vi "Get Class Plugin Parent.vi"(8 "error in (no error)":errorcluster, 11 "LV Class Path":path) -> (0 "error out":errorcluster, 1 "object":refnum<class>, 2 "Qualified Name":string, 3 "Valid":bool)   [LabVIEW 2021, in "Channel.lvlib"]
uses:
  Channel.lvlib
  Channel/Channel_class/Channel.lvclass
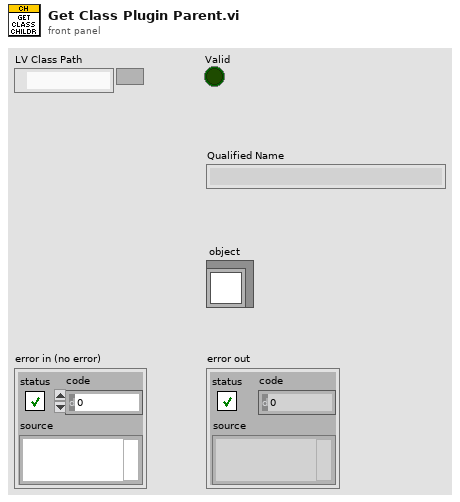
[diagram p1: front panel]
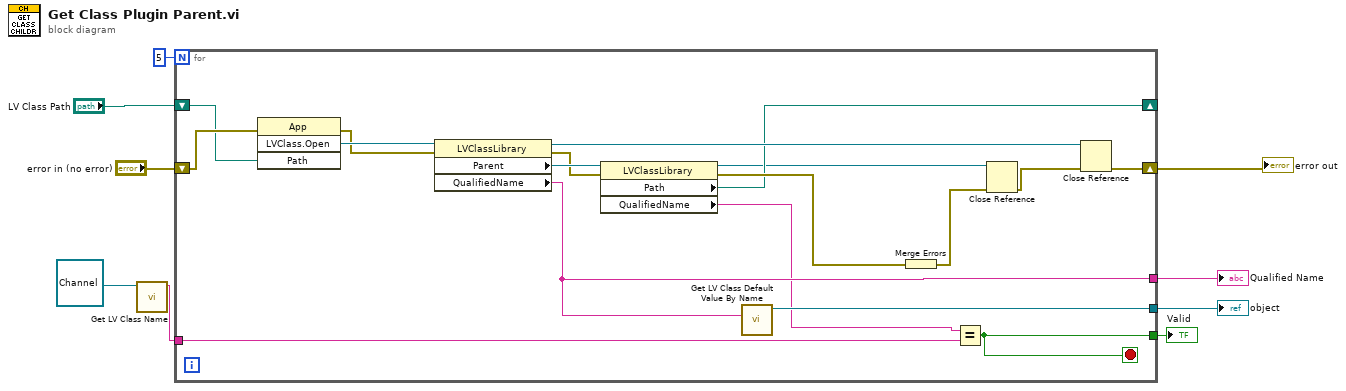
[diagram p0: block diagram]
diagram:
  n1 = call <vilib>:"Get LV Class Name.vi"("object"=refnum<class "Channel.lvclass"> refnum ("Channel.lvlib:Channel")) -> ("class name"=w3:string)  [unwired: 9 in, 1 out]
  n2 = for {
    N: 5 -> [_]
    tunnel: [w11] -> w7
    tunnel: [w16] -> w4
    shift-right: [w19] -> w6
    shift-left: "error in (no error)" -> [w26]
    shift-right: [w15] -> _
    shift-left: "LV Class Path" -> [w25]
    tunnel: w3 -> [w13]
    tunnel: [w12] -> w2
    stop <- w12 stop-if-true
    n3 = invoke on="Invoke Node" class="App" method="LVClass.Open"(error in=w26, "Path"=w25) -> (error out=w24:errorcluster, "LVClass.Open"=w27:refnum<vi>)  [unwired: 2 in, 2 out]
    n4 = property on="Property Node" class="LVClassLibrary"(reference=w27, error in=w24) -> (reference out=w23:refnum<vi>, error out=w20:errorcluster, "Parent"=w21:refnum<vi>, "QualifiedName"=w11:string)
    n5 = property class="LVClassLibrary"(reference=w21, error in=w20) -> (reference out=w14:refnum<vi>, error out=w18:errorcluster, "Path"=w15:path, "QualifiedName"=w10:string)
    n6 = call <vilib>:"Get LV Class Default Value By Name.vi"("class name"=w11) -> ("object"=w16:refnum<class>)  [unwired: 9 in, 1 out]
    n7 = Merge Errors(w18) -> (w17:errorcluster)
    n8 = Equal?(x=w10, y=w13) -> (x = y?=w12:bool)
    n9 = Close Reference(reference=w14, error in (no error)=w17) -> (error out=w22:errorcluster)
    n10 = Close Reference(reference=w23, error in (no error)=w22) -> (error out=w19:errorcluster)
  }
  "error out" <- w6
  "Qualified Name" <- w7
  "object" <- w4
  "Valid" <- w2
